vi "set Sweep Point.vi"(8 "error in (no error)":errorcluster, 10 "Sweep Point":u32, 11 "FSV-40N in":refnum<class "FSV-40N.lvclass">) -> (0 "error out":errorcluster, 3 "FSV-40N out":refnum<class "FSV-40N.lvclass">)   [LabVIEW 2023, in "Spectrum Analyzer.lvlib" / "FSV-40N.lvclass"]
uses:
  FSV-40N.lvclass
  FSV-40N.lvclass/FSV-40N.ctl
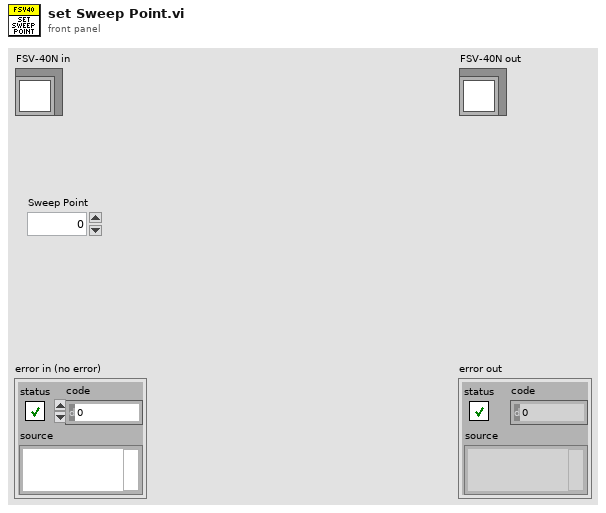
[diagram p1: front panel]
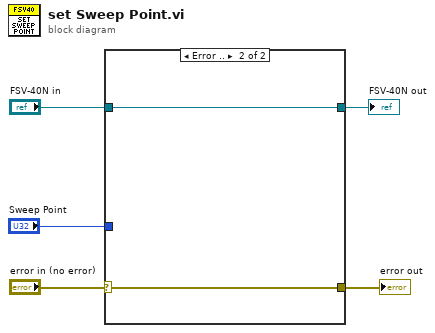
[diagram p0: block diagram]
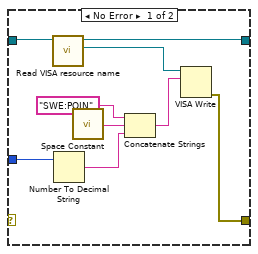
[diagram p2: hidden frame]
diagram:
  n1 = case shown="Error .." "error in (no error)" {
    selector: "error in (no error)" -> [_ w15]
    tunnel: "FSV-40N in" -> [w14 w16]
    tunnel: [w6 w15] -> w3
    tunnel: [w7 w16] -> w2
    tunnel: "Sweep Point" -> [w10 _]
    frame No Error {
      n2 = call "Read VISA resource name.vi"("FSV-40N in"=w14) -> ("VISA resource name"=w13:refnum<visa-resource-name>, "FSV-40N out"=w7:refnum<class "FSV-40N.lvclass">)  [unwired: 8 in, 1 out]
      n3 = Number To Decimal String(number=w10) -> (decimal integer string=w9:string)  [unwired: 1 in]
      n4 = call <vilib>:"Space Constant.vi"() -> ("String"=w11:string)
      n5 = Concatenate Strings("SWE:POIN" ("write buffer"), w11, w9) -> (w8:string)
      n6 = VISA Write(VISA resource name=w13, write buffer=w8) -> (error out=w6:errorcluster)  [unwired: 1 in, 2 out]
    }
    frame Error {
    }
  }
  "error out" <- w3
  "FSV-40N out" <- w2
